vi "Hide SubVI Labels.vi"(8 "error in":errorcluster, 10 "Project Root Folder":path, 11 "Project Manager in":refnum<class "Project Manager.lvclass">) -> (0 "error out":errorcluster, 3 "Project Manager out":refnum<class "Project Manager.lvclass">)   [LabVIEW 2026, in "Project Manager.lvclass"]
doc: "This VI iterates through all VIs in the project and hides Labels of Subvis in the block diagram. Additionally, it cleans up the block diagram."
uses:
  Project Manager.lvclass
  Project Manager.lvclass/Project Manager.ctl
  <vilib>/Utility/traverseref.llb/TRef TravTarget.ctl
  Interfaces/ILogger/ILogger Messages/Log Msg/Log Msg.lvclass/Log Msg.ctl
  <vilib>/ActorFramework/Message Enqueuer/Message Enqueuer.lvclass/Message Enqueuer.ctl
  <vilib>/ActorFramework/Message Enqueuer/Enqueue.vi
  Interfaces/ILogger/ILogger Messages/Log Msg/Log Msg.lvclass
  <vilib>/ActorFramework/Message Priority Queue/Priority Enqueue.vi
  <userlib>/_OpenG.lib/file/file.llb/openg_file.lvlib
  <vilib>/Utility/traverseref.llb/VI Scripting - Traverse.lvlib
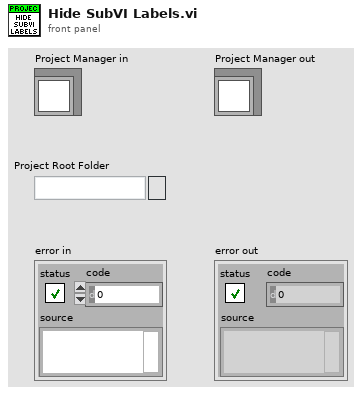
[diagram p1: front panel]
types:
  T1 = typedef "TRef TravTarget.ctl" = enum16{"FP", "BD", "Other"}
  T2 = typedef "Log Entry--cluster.ctl" = cluster{"Time":timestamp, "Message":string}
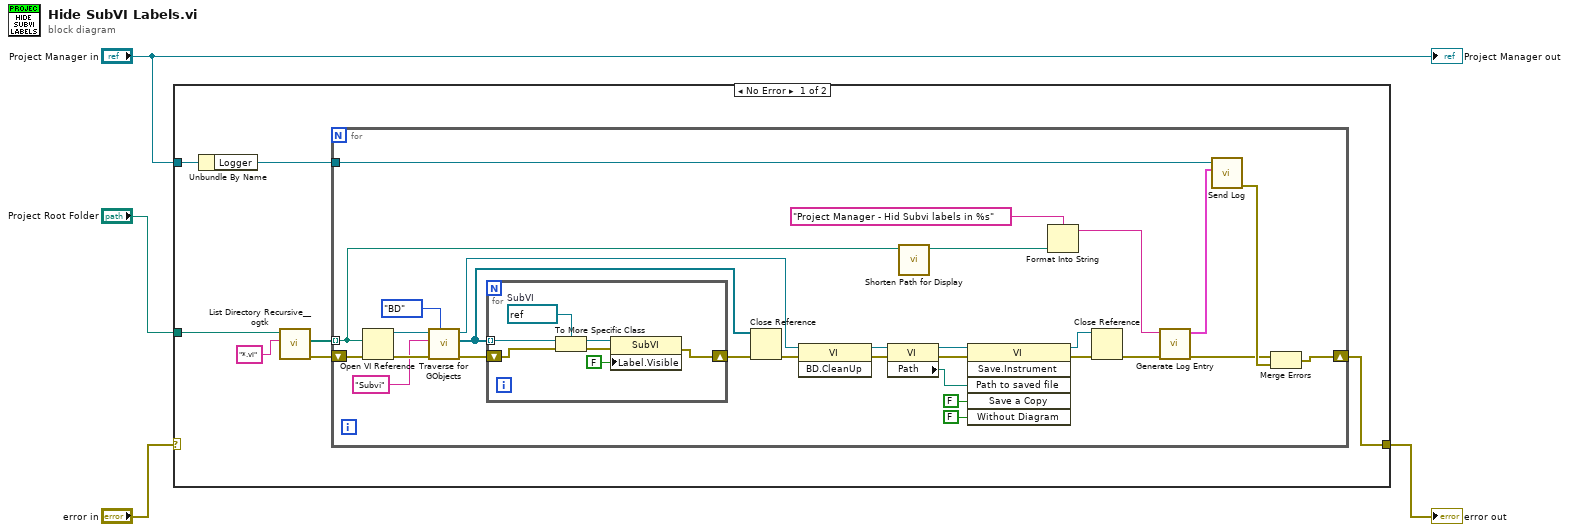
[diagram p0: block diagram]
diagram:
  n1 = case shown="No Error" "error in" {
    selector: "error in" -> [_ w48]
    tunnel: "Project Root Folder" -> [w8 _]
    tunnel: "Project Manager in" -> [w6 _]
    tunnel: [w10 w48] -> w3
    frame No Error {
      n2 = Unbundle By Name(w6) -> ("Logger"=w5:refnum<class "Message Enqueuer.lvclass">)
      n3 = call <userlib>:"List Directory Recursive__ogtk.vi"("pattern"="*.vi", "Path"=w8) -> ("error out"=w11:errorcluster, "file paths"=w7:path[])  [unwired: 6 in, 2 out]
      n4 = for {
        tunnel: w7 -> [w16] mode=indexing
        shift-right: [w34] -> w10
        shift-left: w11 -> [w40]
        tunnel: w5 -> [w18]
        n5 = Open VI Reference(vi path=w16, error in (no error)=w40) -> (vi reference=w28:refnum<vi>, error out=w39:errorcluster)  [unwired: 4 in]
        n6 = call <vilib>:"Traverse for GObjects.vi"("Traverse Target"=TRef_TravTarget."BD", "error in (no error)"=w39, "Class Name"="Subvi", "VI Refnum"=w28) -> ("error out"=w38:errorcluster, "References"=w25:refnum<vi>[], "dup VI Refnum"=w13:refnum<vi>)  [unwired: 4 in, 1 out]
        n7 = for {
          tunnel: w25 -> [w44] mode=indexing
          shift-right: [w45] -> w37
          shift-left: w38 -> [w47]
          w43 = refnum<vi> refnum  # SubVI
          n8 = To More Specific Class(target class=w43, reference=w44, error in=w47) -> (specific class reference=w42:refnum<vi>, error out=w46:errorcluster)
          n9 = property class="SubVI"(reference=w42, error in=w46, "Label.Visible"=FALSE) -> (error out=w45:errorcluster)  [unwired: 1 out]
        }
        n10 = Close Reference(reference=w25, error in (no error)=w37) -> (error out=w30:errorcluster)
        n11 = invoke class="VI" method="BD.CleanUp"(reference=w13, error in=w30) -> (reference out=w12:refnum<vi>, error out=w29:errorcluster)  [unwired: 1 in, 1 out]
        n12 = property class="VI"(reference=w12, error in=w29) -> (reference out=w24:refnum<vi>, error out=w36:errorcluster, "Path"=w23:path)
        n13 = call "Shorten Path for Display.vi"("Path"=w16) -> ("Shortened Path"=w15:path)  [unwired: 10 in]
        n14 = invoke class="VI" method="Save.Instrument"(reference=w24, error in=w36, "Path to saved file"=w23, "Save a Copy"=FALSE, "Without Diagram"=FALSE) -> (reference out=w20:refnum<vi>, error out=w35:errorcluster)  [unwired: 1 in, 4 out]
        n15 = Format Into String(format string="Project Manager - Hid Subvi labels in %s", w15) -> (resulting string=w17:string)  [unwired: 2 in, 1 out]
        n16 = Close Reference(reference=w20, error in (no error)=w35) -> (error out=w32:errorcluster)
        n17 = call "Generate Log Entry.vi"("error in"=w32, "Message"=w17) -> ("error out"=w31:errorcluster, "Log Entry"=w14:T2)  [unwired: 8 in]
        n18 = call "Send Log.vi"("Log Entry"=w14, "Message Enqueuer"=w18) -> ("error out"=w33:errorcluster)  [unwired: 8 in, 1 out]
        n19 = Merge Errors(w31, w33) -> (w34:errorcluster)
      }
    }
    frame Error {
      # "Pass error without further actions."
    }
  }
  "error out" <- w3
  "Project Manager out" <- "Project Manager in"
